vi "Test Open Twice Does Not Leak.vi"() -> ()   [LabVIEW 2019, in "Instrument.lvlib" / "Instrument.lvclass"]
uses:
  Instrument.lvclass
  Instrument.lvclass/Instrument.ctl
  <userlib>/LevyLab/RemoteControl/RemoteControl/RemoteControl.lvclass/RemoteControl.ctl
  <userlib>/LevyLab/RemoteControl/RemoteControl/RemoteControl.lvclass
panel:
  out "Connected=F after close":bool
  out "Connected=T after open":bool
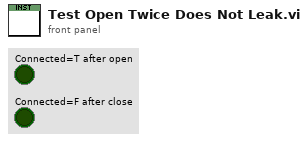
[diagram p1: front panel]
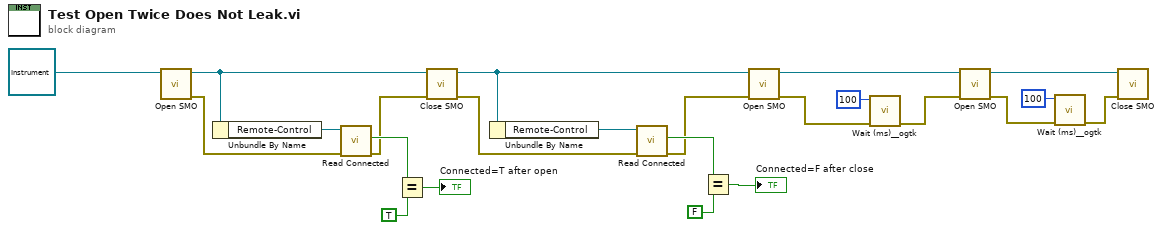
[diagram p0: block diagram]
diagram:
  n1 = call "Open SMO.vi"("Instrument in"=refnum<class "Instrument.lvclass"> refnum) -> ("error out"=w8:errorcluster, "Instrument out"=w22:refnum<class "Instrument.lvclass">)  [unwired: 9 in]
  n2 = Unbundle By Name(w22) -> ("Remote-Control"=w7:refnum<class "RemoteControl.lvclass">)
  n3 = call <userlib>:"Read Connected.vi"("error in (no error)"=w8, "RemoteControl in"=w7) -> ("error out"=w12:errorcluster, "Connected?"=w21:bool)  [unwired: 7 in, 1 out]
  n4 = Equal?(x=w21, y=TRUE) -> (x = y?=→"Connected=T after open":bool)
  n5 = call "Close SMO.vi"("error in (no error)"=w12, "Instrument in"=w22) -> ("error out"=w11:errorcluster, "Instrument out"=w15:refnum<class "Instrument.lvclass">)  [unwired: 8 in]
  n6 = Unbundle By Name(w15) -> ("Remote-Control"=w9:refnum<class "RemoteControl.lvclass">)
  n7 = call <userlib>:"Read Connected.vi"("error in (no error)"=w11, "RemoteControl in"=w9) -> ("error out"=w10:errorcluster, "Connected?"=w18:bool)  [unwired: 7 in, 1 out]
  n8 = Equal?(x=w18, y=FALSE) -> (x = y?=→"Connected=F after close":bool)
  n9 = call "Open SMO.vi"("error in (no error)"=w10, "Instrument in"=w15) -> ("error out"=w6:errorcluster, "Instrument out"=w14:refnum<class "Instrument.lvclass">)  [unwired: 8 in]
  n10 = call <userlib>:"Wait (ms)__ogtk.vi"("error in (no error)"=w6, "milliseconds to wait"=u32 100) -> ("error out"=w5:errorcluster)  [unwired: 8 in, 1 out]
  n11 = call "Open SMO.vi"("error in (no error)"=w5, "Instrument in"=w14) -> ("error out"=w2:errorcluster, "Instrument out"=w13:refnum<class "Instrument.lvclass">)  [unwired: 8 in]
  n12 = call <userlib>:"Wait (ms)__ogtk.vi"("error in (no error)"=w2, "milliseconds to wait"=u32 100) -> ("error out"=w1:errorcluster)  [unwired: 8 in, 1 out]
  n13 = call "Close SMO.vi"("error in (no error)"=w1, "Instrument in"=w13) -> ()  [unwired: 8 in, 2 out]
